vi "Connect.vi"(11 "pHostWin":u32) -> (0 "error out":errorcluster, 2 "function return":i32, 3 "pHostWin out":u32)   [LabVIEW 2011, in "HID_ARZ.lvlib"]
uses:
  HID_ARZ.lvlib
  <userlib>/HID_ARZ/mcHID.dll
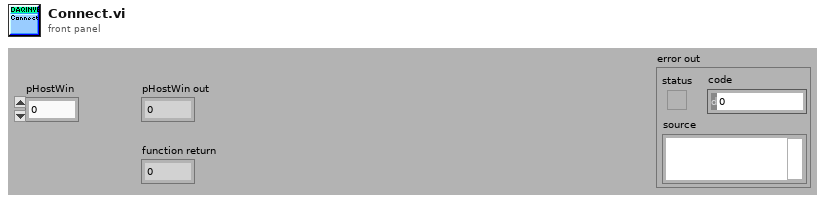
[diagram p1: front panel]
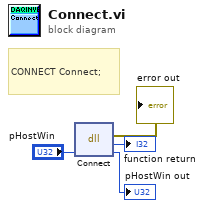
[diagram p0: block diagram]
diagram:
  # "CONNECT Connect;"
  n1 = dll-call lib="C:/Program Files (x86)/National Instruments/LabVIEW 2017/user.lib/HID_ARZ/mcHID.dll" fn="Connect"("pHostWin"="pHostWin") -> (error out=→"error out":errorcluster, "return type"=→"function return":i32, "pHostWin"=→"pHostWin out":u32)  [unwired: 3 in, 1 out]
